vi "IMU Functions.vi"() -> ()   [LabVIEW 2027]
uses:
  <vilib>/MRC/MrcLib/VIs/IMU/IMU Get Euler Angle Flat.vi
  <vilib>/MRC/MrcLib/VIs/IMU/IMU Get Yaw Flat.vi
  <vilib>/MRC/MrcLib.lvlib
panel:
  out "yaw":dbl(graph)
  out "acceleration":cluster{"x":dbl, "y":dbl, "z":dbl}(graph)
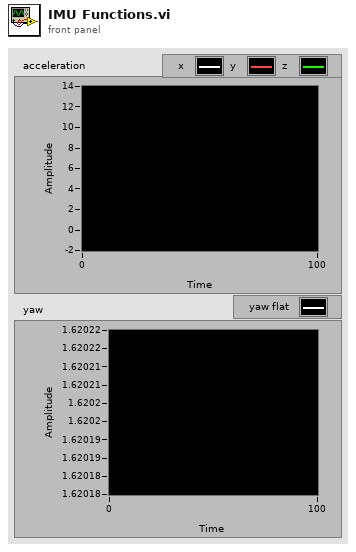
[diagram p1: front panel]
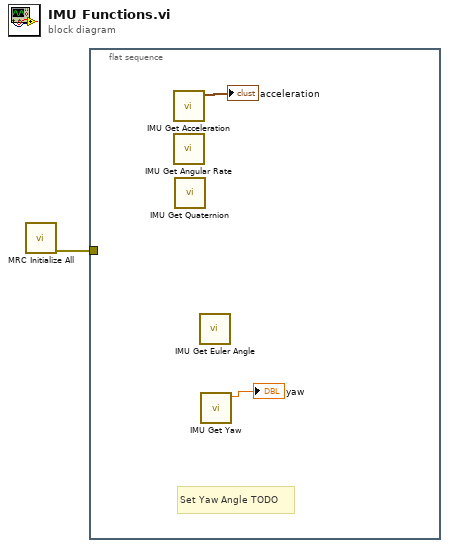
[diagram p0: block diagram]
diagram:
  n1 = call <vilib>:"MRC Initialize All.vi"() -> ("error out"=w1:errorcluster)  [unwired: 11 in]
  n2 = flat-sequence {
    tunnel: w1 -> [_]
    frame #0 {
      # "Set Yaw Angle TODO"
      n3 = call <vilib>:"IMU Get Acceleration.vi"() -> ("acceleration"=→"acceleration":cluster{"x":dbl, "y":dbl, "z":dbl})  [unwired: 9 in, 2 out]
      n4 = call <vilib>:"IMU Get Angular Rate.vi"() -> ()  [unwired: 9 in, 3 out]
      n5 = call <vilib>:"IMU Get Quaternion.vi"() -> ()  [unwired: 9 in, 3 out]
      n6 = call-poly <vilib>:"IMU Get Euler Angle.vi"() -> ()  [unwired: 9 in, 3 out]
      n7 = call-poly <vilib>:"IMU Get Yaw.vi"() -> ("yaw"=→"yaw":dbl)  [unwired: 9 in, 2 out]
    }
  }
